vi "TestSubpanel.vi"(11 "error in":errorcluster) -> (15 "error out":errorcluster)   [LabVIEW 2016, in "SubpanelTests.lvlib"]
doc: "Test Subpanel"
uses:
  SubpanelTests.lvlib
  APIs/Stimulus/ControlValue/ValueSignalByPathString.vi
  APIs/Stimulus/VI/MakeVIFrontMost.vi
  APIs/Stimulus/ControlValue/ValueSignalLatchBooleanString.vi
  APIs/Stimulus/VI/CloseVI.vi
  <vilib>/addons/_JKI Toolkits/Caraya/classes/Test/Test.lvclass
  Drona.lvlib
  APIs/Stimulus/ControlValue/ControlValue.lvlib
  APIs/Stimulus/VI/VI.lvlib
panel:
  # "SUBPANEL TESTS"
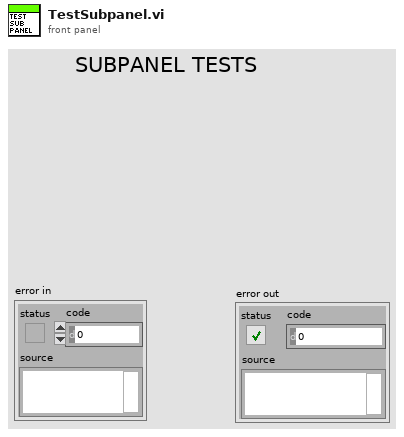
[diagram p1: front panel]
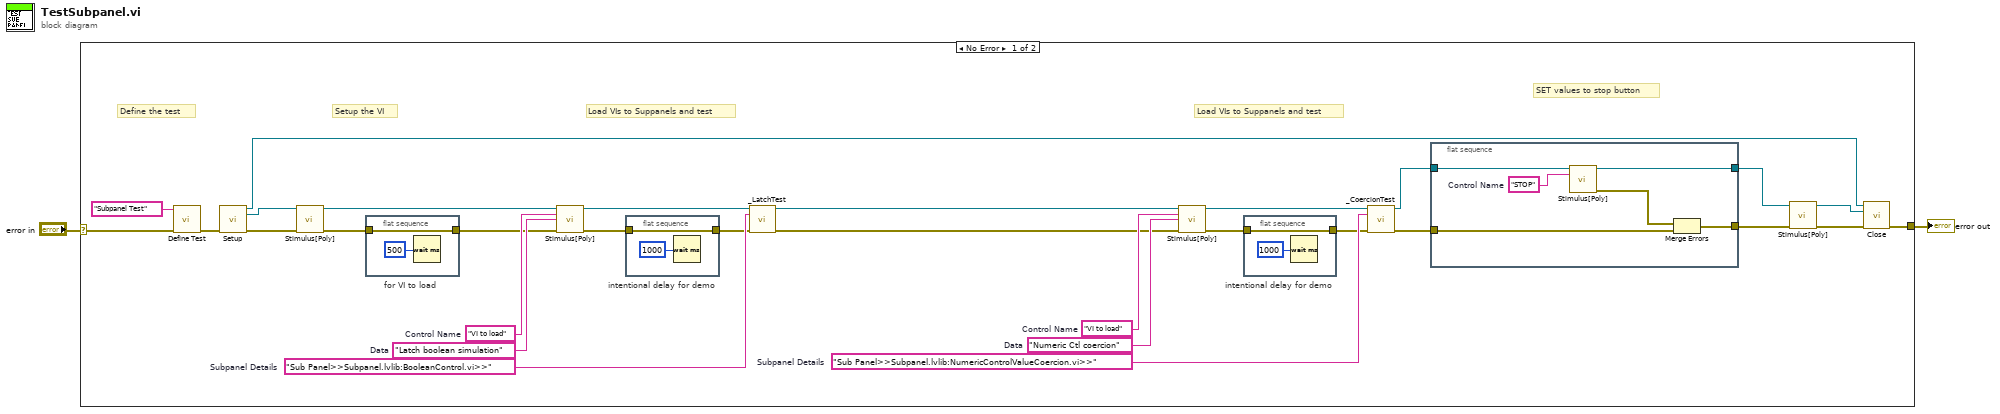
[diagram p0: block diagram]
diagram:
  n1 = case shown="No Error" "error in" {
    selector: "error in" -> [w7 w45]
    tunnel: [w8 w45] -> w2
    frame No Error {
      w24 = "Sub Panel>>Subpanel.lvlib:BooleanControl.vi>>"  # Subpanel Details
      w27 = "Latch boolean simulation"  # Data
      w26 = "VI to load"  # Control Name
      w28 = "Sub Panel>>Subpanel.lvlib:NumericControlValueCoercion.vi>>"  # Subpanel Details
      w30 = "Numeric Ctl coercion"  # Data
      w31 = "VI to load"  # Control Name
      # "Load VIs to Suppanels and test"
      # "Load VIs to Suppanels and test"
      # "SET values to stop button"
      # "Setup the VI"
      # "Define the test"
      n2 = call <vilib>:"Define Test.vi"("error in (no error)"=w7, "Label (VI Title)"="Subpanel Test") -> ("error out"=w14:errorcluster)  [unwired: 8 in, 1 out]
      n3 = call "Setup.vi"("error in"=w14) -> ("Application Ref"=w9:refnum<vi>, "VI Reference Out"=w11:refnum<vi>, "error out"=w13:errorcluster)  [unwired: 12 in]
      n4 = call-poly "Stimulus[Poly].vi"("VI Reference In"=w11, "error in"=w13) -> ("VI Reference Out"=w10:refnum<vi>, "error out"=w12:errorcluster)  [unwired: 12 in]
      n5 = flat-sequence "for VI to load" {
        tunnel: w12 -> [w33]
        tunnel: [w33] -> w15
        frame #0 {
          n6 = Wait (ms)(milliseconds to wait=u32 500) -> ()  [unwired: 1 out]
        }
      }
      n7 = call-poly "Stimulus[Poly].vi"("VI Reference In"=w10, "Control Path"=w26, "Value (Signaling)"=w27, "error in"=w15) -> ("VI Reference Out"=w25:refnum<vi>, "error out"=w19:errorcluster)  [unwired: 10 in]
      n8 = flat-sequence "intentional delay for demo" {
        tunnel: w19 -> [w37]
        tunnel: [w37] -> w18
        frame #0 {
          n9 = Wait (ms)(milliseconds to wait=u32 1000) -> ()  [unwired: 1 out]
        }
      }
      n10 = call "_LatchTest.vi"("VI Reference In"=w25, "Subpanel Details"=w24, "error in"=w18) -> ("VI Reference Out"=w23:refnum<vi>, "error out"=w22:errorcluster)  [unwired: 11 in]
      n11 = call-poly "Stimulus[Poly].vi"("VI Reference In"=w23, "Control Path"=w31, "Value (Signaling)"=w30, "error in"=w22) -> ("VI Reference Out"=w29:refnum<vi>, "error out"=w17:errorcluster)  [unwired: 10 in]
      n12 = flat-sequence "intentional delay for demo" {
        tunnel: w17 -> [w35]
        tunnel: [w35] -> w16
        frame #0 {
          n13 = Wait (ms)(milliseconds to wait=u32 1000) -> ()  [unwired: 1 out]
        }
      }
      n14 = call "_CoercionTest.vi"("VI Reference In"=w29, "Subpanel Details"=w28, "error in"=w16) -> ("VI Reference Out"=w20:refnum<vi>, "error out"=w21:errorcluster)  [unwired: 11 in]
      n15 = flat-sequence {
        tunnel: [w43] -> w6
        tunnel: [w44] -> w4
        tunnel: w21 -> [w40]
        tunnel: w20 -> [w39]
        frame #0 {
          w41 = "STOP"  # Control Name
          n16 = call-poly "Stimulus[Poly].vi"("VI Reference In"=w39, "Control Path"=w41) -> ("VI Reference Out"=w44:refnum<vi>, "error out"=w42:errorcluster)  [unwired: 12 in]
          n17 = Merge Errors(w42, w40) -> (w43:errorcluster)
        }
      }
      n18 = call-poly "Stimulus[Poly].vi"("VI Reference In"=w4, "error in"=w6) -> ("VI Reference Out"=w3:refnum<vi>, "error out"=w5:errorcluster)  [unwired: 12 in]
      n19 = call "Close.vi"("Application Ref"=w9, "VI Reference"=w3, "error in"=w5) -> ("error out"=w8:errorcluster)  [unwired: 12 in]
    }
    frame Error {
    }
  }
  "error out" <- w2
